vi "Body.vi"() -> ()   [LabVIEW 2013]
uses:
  <vilib>/Utility/miscctls.llb/LVPointTypeDef.ctl
  Globals/Global VI.vi
panel:
  out "Access Levels":i32[](array[numeric])
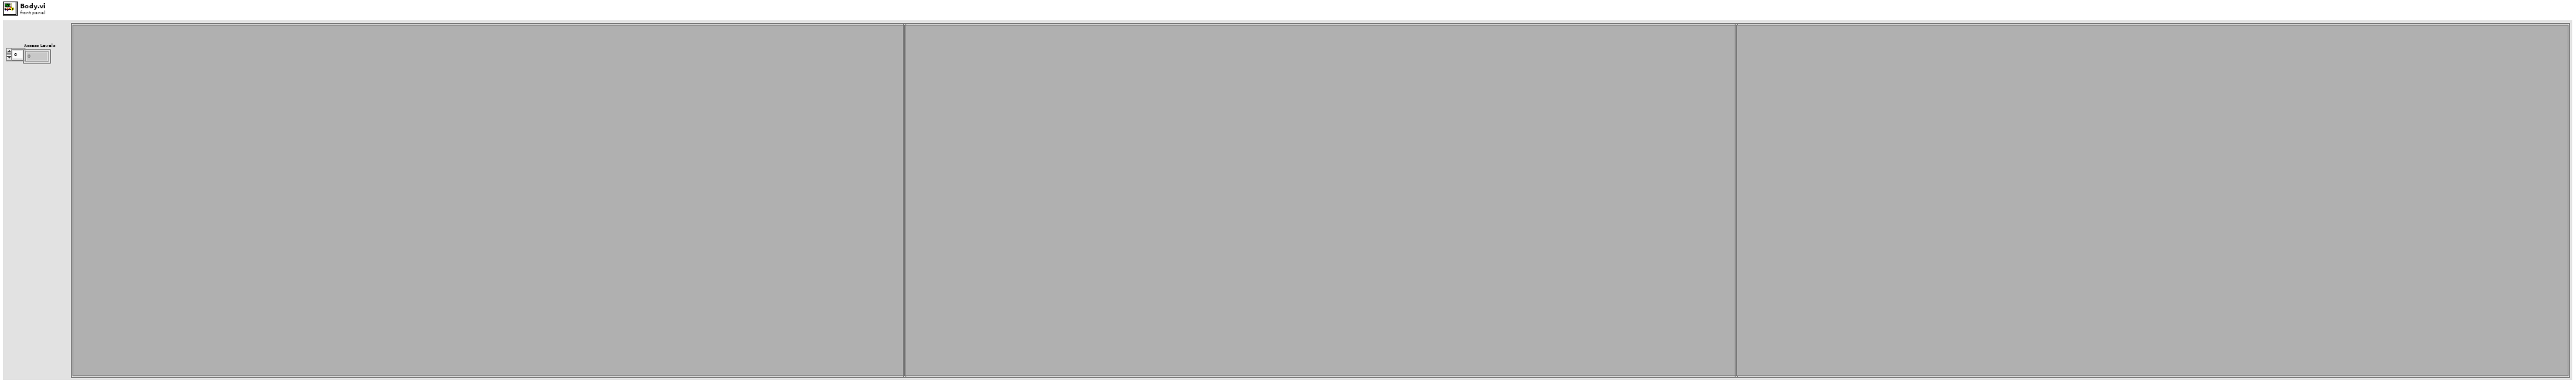
[diagram p1: front panel]
types:
  T1 = typedef "LVPointTypeDef.ctl" = cluster{"Horizontal":i16, "Vertical":i16}
  T2 = enum32{"Bad", "Idle", "Run top level", "Running"}
  T3 = enum8{"Enabled", "Disabled", "Disabled and Grayed Out"}
  T4 = enum16{"Always On", "Always Off", "Off While Running"}
  T5 = typedef "LVAllMonitorsDisplayTypeDef.ctl" = cluster{"Bounds":cluster{"Left":i16, "Top":i16, "Right":i16, "Bottom":i16}, "Depth":i16}[]
  T6 = typedef "LVRectTypeDef.ctl" = cluster{"Left":i16, "Top":i16, "Right":i16, "Bottom":i16}
  T7 = cluster{"Bounds":cluster{"Left":i16, "Top":i16, "Right":i16, "Bottom":i16}, "Depth":i16}
  T8 = typedef "LVBoundsTypeDef.ctl" = cluster{"Width":u32, "Height":u32}
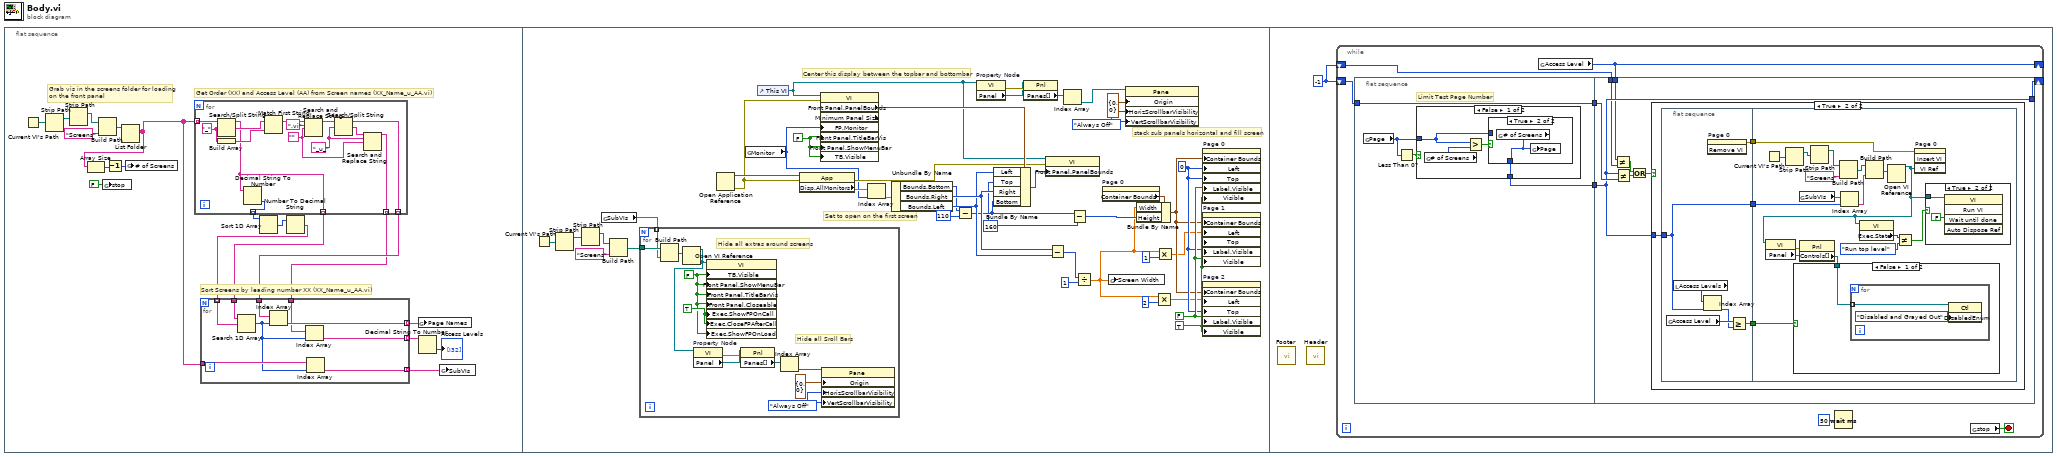
[diagram p0: block diagram]
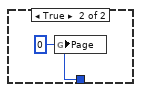
[diagram p3: hidden frame]
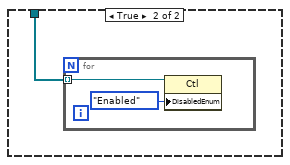
[diagram p6: hidden frame]
diagram:
  n1 = flat-sequence {
    frame #0 {
      # "Get Order (XX) and Access Level (AA) from Screen names (XX_Name_u_AA.vi)"
      # "Sort Screens by leading number XX (XX_Name_u_AA.vi)"
      # "Grab vis in the screens folder for loading\non the front panel"
      n2 = Current VI's Path() -> (path=w18:path)
      n3 = Strip Path(path=w18) -> (stripped path=w16:path)  [unwired: 1 out]
      n4 = Strip Path(path=w16) -> (stripped path=w15:path)  [unwired: 1 out]
      n5 = Build Path(base path=w15, name or relative path="Screens") -> (appended path=w17:path)
      n6 = global write "Global VI.vi" "stop"(FALSE ("stop")) -> ()
      n7 = List Folder(path=w17) -> (filenames=w2:string[])  [unwired: 3 in, 3 out]
      n8 = Array Size(array=w2) -> (size(s)=w13:i32)
      n9 = Decrement(x=w13) -> (x-1=w14:i32)
      n10 = global write "Global VI.vi" "# of Screens"(w14) -> ()
      n11 = for {
        tunnel: [w40] -> w6 mode=indexing
        tunnel: [w31] -> w10 mode=indexing
        tunnel: w2 -> [w32] mode=indexing
        tunnel: [w30] -> w9 mode=indexing
        tunnel: [w29] -> w4 mode=indexing
        w34 = "_" ("search string/char (-)")
        w38 = "_u_" ("search string/char (-)")
        w37 = ""
        n12 = Search/Split String(string=w32, search string/char (-)=w34) -> (substring before match=w31:string, match + rest of string=w36:string)  [unwired: 1 in, 1 out]
        n13 = Build Array(w34) -> (w33:string[])
        n14 = Decimal String To Number(string=w31) -> (number=w30:i32)  [unwired: 2 in, 1 out]
        n15 = Match First String(2:w33, 3:w36) -> (1:w35:string)  [unwired: 1 out]
        n16 = Search and Replace String(input string=w35, search string=".vi", replace string=w37) -> (result string=w41:string)  [unwired: 5 in, 3 out]
        n17 = Search/Split String(string=w41, search string/char (-)=w38) -> (substring before match=w40:string, match + rest of string=w39:string)  [unwired: 1 in, 1 out]
        n18 = Search and Replace String(input string=w39, search string=w38, replace string=w37) -> (result string=w29:string)  [unwired: 5 in, 3 out]
      }
      n19 = Sort 1D Array(array=w9) -> (sorted array=w8:i32[])
      n20 = Number To Decimal String(number=w8) -> (decimal integer string=w7:string[])  [unwired: 1 in]
      n21 = for {
        tunnel: w10 -> [w28]
        tunnel: w7 -> [w27] mode=indexing
        tunnel: w6 -> [w26]
        tunnel: [w25] -> w5 mode=indexing
        tunnel: w4 -> [w24]
        tunnel: [w23] -> w3 mode=indexing
        tunnel: w2 -> [w22]
        tunnel: [w20] -> w1 mode=indexing
        n22 = Search 1D Array(1D array=w28, element=w27) -> (index of element=w21:i32)  [unwired: 1 in]
        n23 = Index Array(array=w26, index=w21) -> (element=w25:string)
        n24 = Index Array(array=w24, index=w21) -> (element=w23:string)
        n25 = Index Array(array=w22, index=w21) -> (element=w20:string)
      }
      n26 = global write "Global VI.vi" "Page Names"(w5) -> ()
      n27 = Decimal String To Number(string=w3) -> (number=→"Access Levels":i32[])  [unwired: 2 in, 1 out]
      n28 = global write "Global VI.vi" "SubVIs"(w1) -> ()
    }
    frame #1 {
      w43 = T4."Always Off" ("Horizontal Scrollbar Visibility")
      w45 = FALSE ("Front Panel Window:Title Bar Visible")
      w76 = TRUE ("Label.Visible")
      w75 = FALSE ("Label.Visible")
      w74 = 0 ("Position:Left")
      w66 = i16 160 ("top")
      # "Set to open on the first screen"
      # "stack sub panels horizontal and fill screen"
      # "Center this display between the topbar and bottombar"
      n29 = Current VI's Path() -> (path=w81:path)
      n30 = Strip Path(path=w81) -> (stripped path=w48:path)  [unwired: 1 out]
      n31 = Strip Path(path=w48) -> (stripped path=w47:path)  [unwired: 1 out]
      n32 = global read "Global VI.vi" "SubVIs"() -> (w51:string[])
      n33 = Build Path(base path=w47, name or relative path="Screens") -> (appended path=w83:path)
      n34 = for {
        tunnel: w83 -> [w94]
        tunnel: w51 -> [w93] mode=indexing
        w91 = T4."Always Off" ("Horizontal Scrollbar Visibility")
        w92 = TRUE ("Execution:Show Front Panel On Call")
        w84 = FALSE ("Tool Bar:Visible")
        # "Hide all extras around screens"
        # "Hide all Sroll Bars"
        n35 = Build Path(base path=w94, name or relative path=w93) -> (appended path=w95:path)
        n36 = Open VI Reference(vi path=w95) -> (vi reference=w85:refnum<vi>)  [unwired: 5 in, 1 out]
        n37 = property on="Property Node" class="VI"(reference=w85) -> (error out=w88:errorcluster, "Panel"=w89:refnum<vi>)  [unwired: 1 in, 1 out]
        n38 = property class="VI"(reference=w85, "TB.Visible"=w84, "Front Panel.ShowMenuBar"=w84, "Front Panel.TitleBarVis"=w84, "Front Panel.Closeable"=w84, "Exec.ShowFPOnCall"=w92, "Exec.CloseFPAfterCall"=w92, "Exec.ShowFPOnLoad"=w84) -> ()  [unwired: 1 in, 2 out]
        n39 = property class="Pnl"(reference=w89, error in=w88) -> ("Panes[]"=w90:refnum<vi>[])  [unwired: 2 out]
        n40 = Index Array "Index Array"(array=w90) -> (element=w86:refnum<vi>)  [unwired: 1 in]
        n41 = property class="Pane"(reference=w86, "Origin"=T1 {"Horizontal"=0, "Vertical"=0}, "HorizScrollbarVisibility"=w91, "VertScrollbarVisibility"=w91) -> ()  [unwired: 1 in, 2 out]
      }
      n42 = Open Application Reference() -> (0:w57:errorcluster, 3:w63:refnum<vi>)  [unwired: 4 in]
      n43 = global read "Global VI.vi" "Monitor"() -> (w50:u16)
      n44 = control-ref of="This VI"() -> (w46:refnum<vi>)
      n45 = property class="App"(reference=w63, error in=w57) -> (error out=w54:errorcluster, "Disp.AllMonitors"=w53:T5)  [unwired: 1 out]
      n46 = property class="VI" props=["Front Panel.PanelBounds", "Minimum Panel Size", "FP.Monitor", "Front Panel.TitleBarVis", "Front Panel.ShowMenuBar", "TB.Visible"](reference=w46, error in=w57, "FP.Monitor"=w50, "Front Panel.TitleBarVis"=w45, "Front Panel.ShowMenuBar"=w45, "TB.Visible"=w45) -> ("Front Panel.PanelBounds"=w56:T6)  [unwired: 3 out]
      n47 = Index Array(array=w53, index=w50) -> (element=w52:T7)
      n48 = Unbundle By Name(w52) -> ("Bounds.Bottom"=w58:i16, "Bounds.Right"=w78:i16, "Bounds.Left"=w77:i16)
      n49 = Subtract(x=w58, y=i16 110) -> (x-y=w67:i16)
      n50 = property on="Property Node" class="VI"(reference=w46) -> (error out=w61:errorcluster, "Panel"=w60:refnum<vi>)  [unwired: 1 in, 1 out]
      n51 = Bundle By Name(cluster=w56, "Left"=w77, "Top"=w66, "Right"=w78, "Bottom"=w67) -> (w55:T6)
      n52 = property class="Pnl"(reference=w60, error in=w61) -> ("Panes[]"=w44:refnum<vi>[])  [unwired: 2 out]
      n53 = property class="VI"(reference=w46, error in=w54, "Front Panel.PanelBounds"=w55) -> ()  [unwired: 2 out]
      n54 = Subtract(x=w78, y=w77) -> (x-y=w79:i16)
      n55 = Index Array "Index Array"(array=w44) -> (element=w64:refnum<vi>)  [unwired: 1 in]
      n56 = Subtract(x=w67, y=w66) -> (x-y=w68:i16)
      n57 = Divide(x=w79, y=i16 1) -> (x/y=w49:dbl)
      n58 = property on="Page 0" class="SubPnl"() -> ("Container Bounds"=w65:T8)  [unwired: 2 in, 2 out]
      n59 = global write "Global VI.vi" "Screen Width"(w49) -> ()
      n60 = property class="Pane"(reference=w64, "Origin"=T1 {"Horizontal"=0, "Vertical"=0}, "HorizScrollbarVisibility"=w43, "VertScrollbarVisibility"=w43) -> ()  [unwired: 1 in, 2 out]
      n61 = Bundle By Name(cluster=w65, "Width"=w49, "Height"=w68) -> (w71:T8)
      n62 = Multiply(x=w49, y=i16 2) -> (x*y=w73:dbl)
      n63 = Multiply(x=w49, y=i16 1) -> (x*y=w70:dbl)
      n64 = property on="Page 0" class="SubPnl"("Container Bounds"=w71, "Left"=w74, "Top"=w74, "Label.Visible"=w75, "Visible"=w76) -> ()  [unwired: 2 in, 2 out]
      n65 = property on="Page 1" class="SubPnl"("Container Bounds"=w71, "Left"=w70, "Top"=w74, "Label.Visible"=w75, "Visible"=w76) -> ()  [unwired: 2 in, 2 out]
      n66 = property on="Page 2" class="SubPnl"("Container Bounds"=w71, "Left"=w73, "Top"=w74, "Label.Visible"=w75, "Visible"=w76) -> ()  [unwired: 2 in, 2 out]
    }
    frame #2 {
      w96 = i16 -1 ("Page")
      n67 = call "Footer.vi"() -> ()  [unwired: 12 in]
      n68 = call "Header.vi"() -> ()  [unwired: 12 in]
      n69 = while {
        shift-right: [w101] -> _
        shift-left: w96 -> [w102]
        shift-right: [w99] -> _
        shift-left: w96 -> [w98]
        stop <- w104 stop-if-true
        n70 = flat-sequence {
          tunnel: [w107] -> w103
          tunnel: w102 -> [w107]
          tunnel: [w105] -> w100
          tunnel: w103 -> [w122]
          tunnel: [w121] -> w101
          tunnel: w100 -> [w121]
          tunnel: w99 -> [w120]
          tunnel: w98 -> [w119]
          frame #0 {
            # "Limit Test Page Number"
            n71 = global read "Global VI.vi" "Page"() -> (w106:i16)
            n72 = Less Than 0?(x=w106) -> (x < 0?=w108:bool)
            n73 = case shown="False" w108 {
              tunnel: w106 -> [w109 _]
              tunnel: [w110 w115] -> w105
              frame False {
                n74 = global read "Global VI.vi" "# of Screens"() -> (w111:i16)
                n75 = Greater?(x=w109, y=w111) -> (0:w112:bool)
                n76 = case shown="True" w112 {
                  tunnel: [w113 w114] -> w110
                  tunnel: w109 -> [w113 _]
                  frame False {
                  }
                  frame True {
                    n77 = global read "Global VI.vi" "# of Screens"() -> (w114:i16)
                    n78 = global write "Global VI.vi" "Page"(w114) -> ()
                  }
                }
              }
              frame True {
                w115 = i16 0 ("Page")
                n79 = global write "Global VI.vi" "Page"(w115) -> ()
              }
            }
          }
          frame #1 {
            n80 = Not Equal?(x=w120, y=w119) -> (x != y?=w116:bool)
            n81 = Not Equal?(x=w121, y=w122) -> (x != y?=w117:bool)
            n82 = Or(x=w116, y=w117) -> (x .or. y?=w118:bool)
            n83 = case shown="True" w118 {
              tunnel: w121 -> [_ w125]
              frame False {
              }
              frame True {
                n84 = flat-sequence {
                  tunnel: [w132] -> w126
                  tunnel: w125 -> [w128]
                  tunnel: [w128] -> w124
                  tunnel: [w130] -> w123
                  tunnel: w126 -> [w142]
                  tunnel: w124 -> [w141]
                  tunnel: w123 -> [w137]
                  frame #0 {
                    n85 = global read "Global VI.vi" "Access Level"() -> (w131:u16)
                    n86 = local read "Access Levels"() -> (w129:i32[])
                    n87 = Index Array(array=w129, index=w128) -> (element=w127:i32)
                    n88 = invoke on="Page 0" class="SubPnl" method="Remove VI"() -> (error out=w132:errorcluster)  [unwired: 3 in, 2 out]
                    n89 = Greater Or Equal?(x=w131, y=w127) -> (x >= y?=w130:bool)
                  }
                  frame #1 {
                    n90 = Current VI's Path() -> (path=w149:path)
                    n91 = Strip Path(path=w149) -> (stripped path=w148:path)  [unwired: 1 out]
                    n92 = global read "Global VI.vi" "SubVIs"() -> (w144:string[])
                    n93 = Strip Path(path=w148) -> (stripped path=w147:path)  [unwired: 1 out]
                    n94 = Build Path(base path=w147, name or relative path="Screens") -> (appended path=w145:path)
                    n95 = Index Array(array=w144, index=w141) -> (element=w143:string)
                    n96 = Build Path(base path=w145, name or relative path=w143) -> (appended path=w146:path)
                    n97 = Open VI Reference(vi path=w146) -> (vi reference=w136:refnum<vi>)  [unwired: 5 in, 1 out]
                    n98 = property class="VI"(reference=w136) -> (error out=w139:errorcluster, "Panel"=w140:refnum<vi>)  [unwired: 1 in, 1 out]
                    n99 = property class="Pnl"(reference=w140, error in=w139) -> ("Controls[]"=w138:refnum<vi>[])  [unwired: 2 out]
                    n100 = case shown="False" w137 {
                      tunnel: w138 -> [w153 w156]
                      frame False {
                        n101 = for {
                          tunnel: w153 -> [w155] mode=indexing
                          n102 = property class="Ctl"(reference=w155, "DisabledEnum"=T3."Disabled and Grayed Out" ("Disabled")) -> ()  [unwired: 1 in, 2 out]
                        }
                      }
                      frame True {
                        n103 = for {
                          tunnel: w156 -> [w158] mode=indexing
                          n104 = property class="Ctl"(reference=w158, "DisabledEnum"=T3."Enabled" ("Disabled")) -> ()  [unwired: 1 in, 2 out]
                        }
                      }
                    }
                    n105 = property class="VI"(reference=w136) -> ("Exec.State"=w134:T2)  [unwired: 1 in, 2 out]
                    n106 = Not Equal?(x=w134, y=T2."Run top level" ("Execution:State")) -> (x != y?=w133:bool)
                    n107 = invoke on="Page 0" class="SubPnl" method="Insert VI"(error in=w142, "VI Ref"=w136) -> ()  [unwired: 2 in, 4 out]
                    n108 = case shown="True" w133 {
                      tunnel: w136 -> [_ w152]
                      frame False {
                      }
                      frame True {
                        n109 = invoke class="VI" method="Run VI"(reference=w152, "Wait until done"=FALSE ("Wait Until Done")) -> ()  [unwired: 3 in, 5 out]
                      }
                    }
                  }
                }
              }
            }
          }
        }
        n110 = global read "Global VI.vi" "Access Level"() -> (w99:u16)
        n111 = Wait (ms)(milliseconds to wait=u32 50) -> ()  [unwired: 1 out]
        n112 = global read "Global VI.vi" "stop"() -> (w104:bool)
      }
    }
  }
